vi "DumpFileWriteData.vi"(10 "Data":dbl[][](array[numeric]), 11 "DumpFileState":T1) -> (3 "DumpFileState out":T1)   [LabVIEW 2025]
uses:
  DumpFileState.ctl
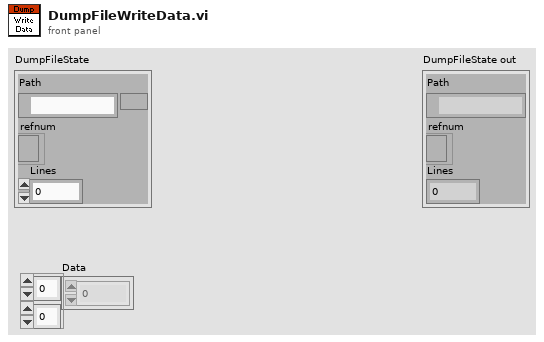
[diagram p1: front panel]
types:
  T1 = typedef "DumpFileState.ctl" = cluster{"Path":path, "refnum":refnum<file>, "Lines":i32}
  T2 = enum16{"big-endian, network order", "native, host order", "little-endian"}
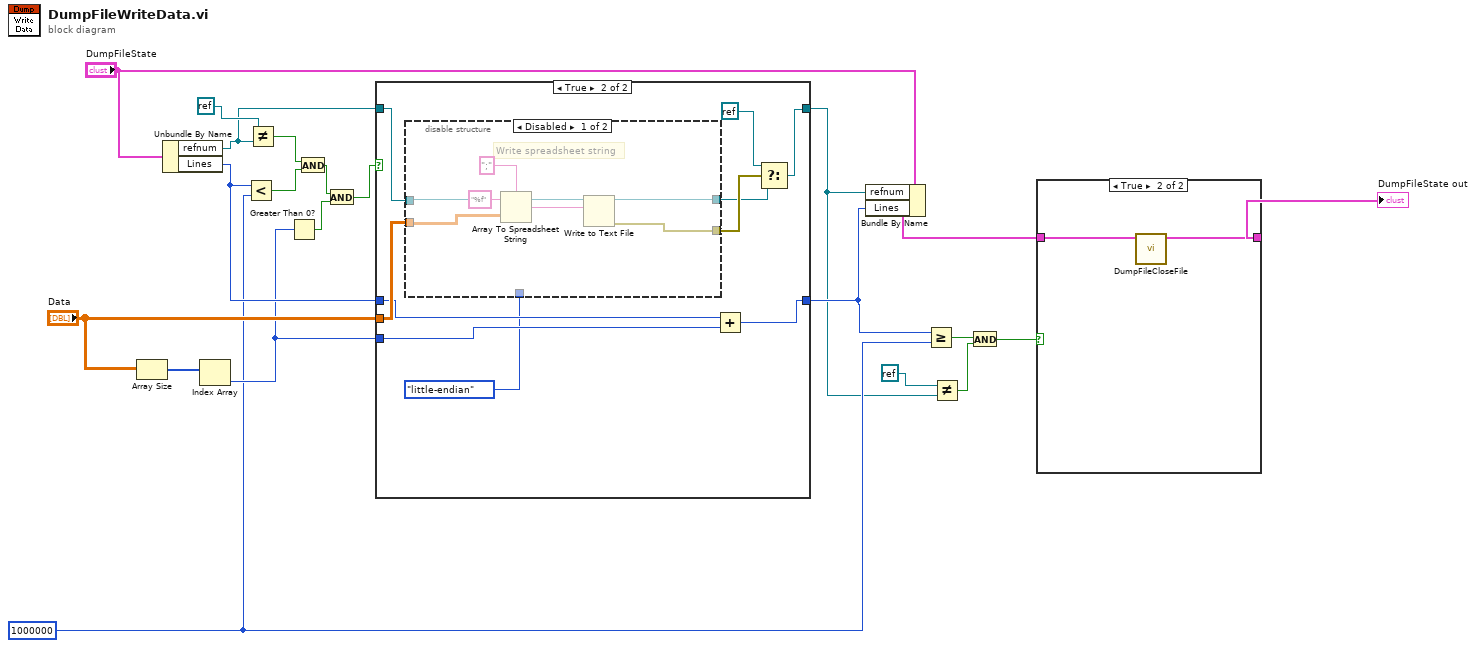
[diagram p0: block diagram]
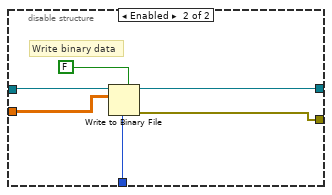
[diagram p4: hidden frame]
diagram:
  w8 = 1000000 ("y")
  n1 = Array Size(array="Data") -> (size(s)=w14:i32[])
  n2 = Unbundle By Name("DumpFileState") -> ("refnum"=w16:refnum<file>, "Lines"=w15:i32)
  n3 = Index Array(array=w14) -> (element=w13:i32)  [unwired: 1 in]
  n4 = Less?(x=w15, y=w8) -> (x < y?=w17:bool)
  n5 = Not Equal?(x=refnum<k0> refnum, y=w16) -> (x != y?=w18:bool)
  n6 = Greater Than 0?(x=w13) -> (x > 0?=w12:bool)
  n7 = And(x=w18, y=w17) -> (x .and. y?=w11:bool)
  n8 = And(x=w11, y=w12) -> (x .and. y?=w10:bool)
  n9 = case shown="True" w10 {
    tunnel: "Data" -> [_ w32]
    tunnel: w16 -> [w23 w33]
    tunnel: [w23 w26] -> w6
    tunnel: w15 -> [w22 w31]
    tunnel: [w22 w30] -> w9
    tunnel: w13 -> [_ w25]
    frame False {
    }
    frame True {
      n10 = disable-structure shown="Disabled" {
        disable-tunnel: w33 -> [w37 w44]
        disable-tunnel: w32 -> [w34 w41]
        disable-tunnel: [w36 w42] -> w29
        disable-tunnel: [w35 w43] -> w27
        disable-tunnel: T2."little-endian" ("byte order (0:big-endian, network order)") -> [_ w45]
        frame Disabled {
          # "Write spreadsheet string"
          n11 = Array To Spreadsheet String(delimiter (Tab)=";", array=w34, 3:"%f" ("format string")) -> (spreadsheet string=w38:string)
          n12 = Write to Text File(file (use dialog)=w37, text=w38) -> (refnum out=w35:refnum<file>, error out=w36:errorcluster)  [unwired: 2 in, 1 out]
        }
        frame Enabled {
          # "Write binary data"
          n13 = Write to Binary File(file (use dialog)=w44, data=w41, 5:FALSE ("prepend array or string size? (T)"), 9:w45) -> (refnum out=w43:refnum<file>, error out=w42:errorcluster)  [unwired: 2 in, 1 out]
        }
      }
      n14 = Add(x=w31, y=w25) -> (x+y=w30:i32)
      n15 = Select(t=refnum<k0> refnum, s=w29, f=w27) -> (s? t:f=w26:refnum<file>)
    }
  }
  n16 = Bundle By Name(cluster="DumpFileState", "refnum"=w6, "Lines"=w9) -> (w2:T1)
  n17 = Greater Or Equal?(x=w9, y=w8) -> (x >= y?=w5:bool)
  n18 = Not Equal?(x=refnum<k0> refnum, y=w6) -> (x != y?=w4:bool)
  n19 = And(x=w5, y=w4) -> (x .and. y?=w3:bool)
  n20 = case shown="True" w3 {
    tunnel: w2 -> [w47 w49]
    tunnel: [w47 w48] -> w1
    frame False {
    }
    frame True {
      n21 = call "DumpFileCloseFile.vi"("DumpFileState"=w49) -> ("DumpFileState out"=w48:T1)  [unwired: 10 in]
    }
  }
  "DumpFileState out" <- w1
